vi "vi_save.vi"() -> ()   [LabVIEW 2014]
panel:
  out "error out":errorcluster
  out "reference out":refnum<vi>
  in  "Without Diagram":bool
  in  "Save a Copy":bool
  in  "Path to Saved File":path
  in  "error in (no error)":errorcluster
  in  "reference":refnum<vi>
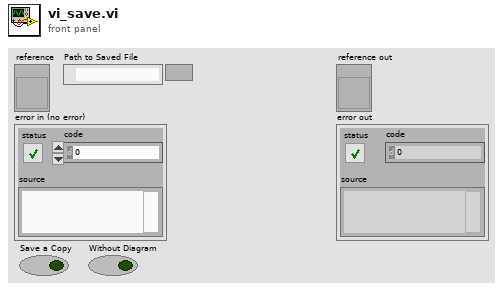
[diagram p1: front panel]
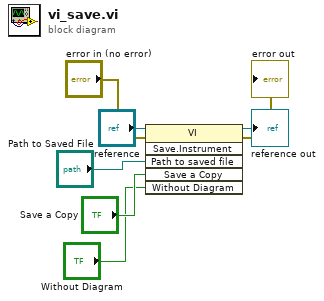
[diagram p0: block diagram]
diagram:
  n1 = invoke class="VI" method="Save.Instrument"(reference="reference", error in="error in (no error)", "Path to saved file"="Path to Saved File", "Save a Copy"="Save a Copy", "Without Diagram"="Without Diagram") -> (reference out=→"reference out":refnum<vi>, error out=→"error out":errorcluster)  [unwired: 1 in, 4 out]
